vi "VIH HelpGen - Get Control Tag.vi"(7 "Separator (.)":string=".", 8 "error in":errorcluster, 9 "Skip Cluster if it's Array element (T)":bool=TRUE, 11 "Ctl Refnum":refnum<vi>) -> (0 "error out":errorcluster, 1 "Label":string, 2 "Control Tag":string, 3 "dup Ctl Refnum":refnum<vi>, 4 "Class Name":string, 5 "Parent Control Tag":string)   [LabVIEW 2014]
doc: "The VI builds a Control Tag of the specified control.\n\n::: VI Helpeks :::\nCopyright (c) 2000-2026 Konstantin Shifershteyn. All rights reserved."
panel:
  # "VI Helpeks\nCopyright (c) 2012-2026 Konstantin Shifershteyn"
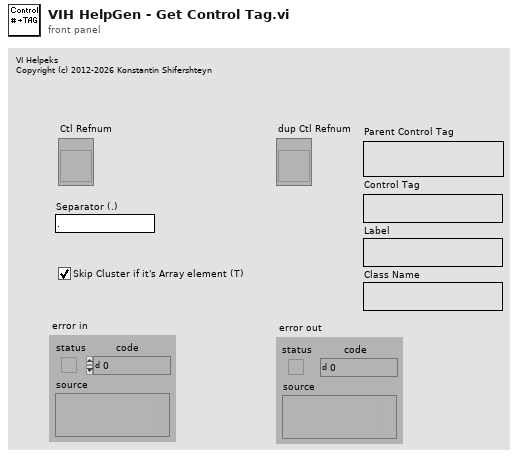
[diagram p1: front panel]
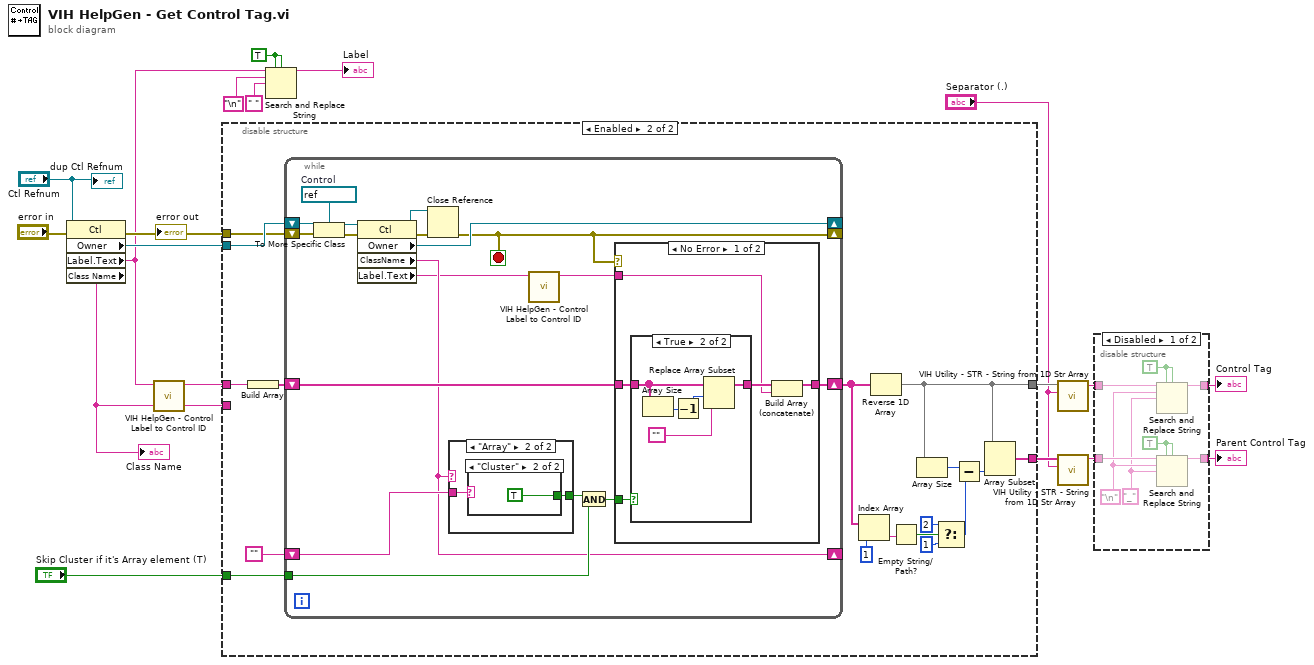
[diagram p0: block diagram]
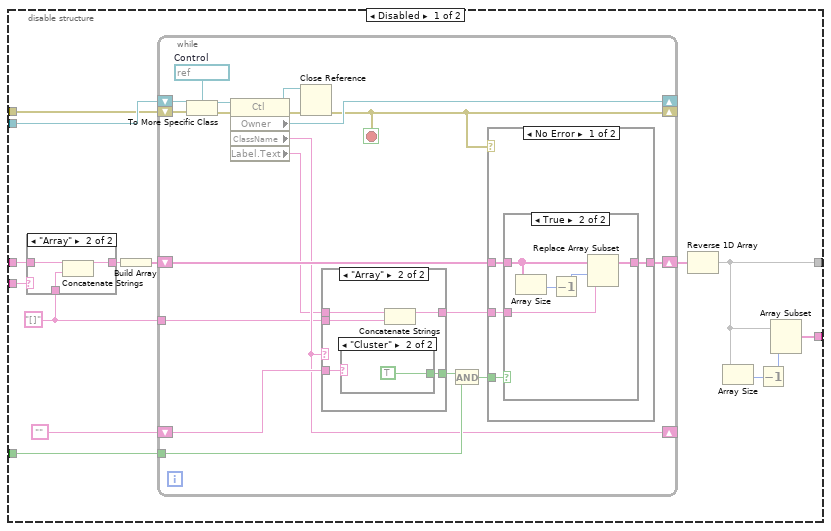
[diagram p3: hidden frame]
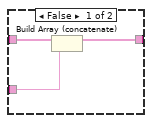
[diagram p7: hidden frame]
diagram:
  w5 = TRUE
  n1 = property class="Ctl"(reference="Ctl Refnum", error in="error in") -> (error out=w17:errorcluster, "Owner"=w18:refnum<vi>, "Label.Text"=w2:string, "Class Name"=w11:string)  [unwired: 1 out]
  "error out" <- w17
  "Class Name" <- w11
  n2 = call "VIH HelpGen - Control Label to Control ID.vi"("Control Name"=w2) -> ("Control ID"=w6:string)  [unwired: 10 in]
  n3 = disable-structure shown="Enabled" {
    disable-tunnel: w18 -> [w33 w93]
    disable-tunnel: w17 -> [w32 w92]
    disable-tunnel: "Skip Cluster if it's Array element (T)" -> [w30 w90]
    disable-tunnel: [w25 w77] -> w14
    disable-tunnel: [w24 w88] -> w13
    disable-tunnel: w6 -> [w23 w87]
    disable-tunnel: w11 -> [w20 _]
    frame Disabled {
      w21 = "[]" ("string")
      n4 = case shown="\"Array\"" w20 {
        tunnel: w23 -> [w34 w37]
        tunnel: [w34 w36] -> w22
        tunnel: w21 -> [_ w35]
        frame Default {
        }
        frame "Array" {
          n5 = Concatenate Strings(w37, w35) -> (w36:string)
        }
      }
      n6 = Build Array(w22) -> (w28:string[])
      n7 = while {
        shift-right: [w42] -> _
        shift-left: w32 -> [w49]
        shift-right: [w53] -> w29
        shift-left: w28 -> [w54]
        shift-right: [w52] -> _
        shift-left: w33 -> [w50]
        shift-right: [w43] -> _
        shift-left: "" -> [w45]
        tunnel: w30 -> [w44]
        tunnel: w21 -> [w38]
        stop <- w42 stop-if-true
        w51 = refnum<vi> refnum  # Control
        n8 = To More Specific Class(target class=w51, reference=w50, error in=w49) -> (specific class reference=w47:refnum<vi>, error out=w48:errorcluster)
        n9 = property class="Ctl"(reference=w47, error in=w48) -> (reference out=w56:refnum<vi>, error out=w55:errorcluster, "Owner"=w52:refnum<vi>, "ClassName"=w43:string, "Label.Text"=w41:string)
        n10 = Close Reference(reference=w56, error in (no error)=w55) -> (error out=w42:errorcluster)
        n11 = case shown="\"Array\"" w43 {
          tunnel: w45 -> [_ w62]
          tunnel: [_ w61] -> w46
          tunnel: w41 -> [w57 w60]
          tunnel: [w57 w59] -> w40
          tunnel: w38 -> [_ w58]
          frame Default {
          }
          frame "Array" {
            n12 = case shown="\"Cluster\"" w62 {
              tunnel: [_ TRUE] -> w61
              frame Default {
              }
              frame "Cluster" {
              }
            }
            n13 = Concatenate Strings(w60, w58) -> (w59:string)
          }
        }
        n14 = And(x=w46, y=w44) -> (x .and. y?=w39:bool)
        n15 = case shown="No Error" w42 {
          tunnel: w54 -> [w65 w76]
          tunnel: w40 -> [w67 _]
          tunnel: [w66 w76] -> w53
          tunnel: w39 -> [w64 _]
          frame No Error {
            n16 = case shown="True" w64 {
              tunnel: w67 -> [w69 w72]
              tunnel: [w68 w71] -> w66
              tunnel: w65 -> [w70 w75]
              frame False {
                n17 = Build Array (concatenate)(w70, w69) -> (w68:string[])
              }
              frame True {
                n18 = Array Size(array=w75) -> (size(s)=w74:i32)
                n19 = Decrement(x=w74) -> (x-1=w73:i32)
                n20 = Replace Array Subset(array=w75, new element=w72, index=w73) -> (w71:string[])
              }
            }
          }
          frame Error {
          }
        }
      }
      n21 = Reverse 1D Array(array=w29) -> (reversed array=w25:string[])
      n22 = Array Size(array=w25) -> (size(s)=w26:i32)
      n23 = Decrement(x=w26) -> (x-1=w27:i32)
      n24 = Array Subset(array=w25, length=w27) -> (w24:string[])  [unwired: 1 in]
    }
    frame Enabled {
      n25 = Build Array(w87) -> (w89:string[])
      n26 = while {
        shift-right: [w97] -> _
        shift-left: w92 -> [w104]
        shift-right: [w108] -> w82
        shift-left: w89 -> [w109]
        shift-right: [w107] -> _
        shift-left: w93 -> [w105]
        shift-right: [w98] -> _
        shift-left: "" -> [w100]
        tunnel: w90 -> [w99]
        stop <- w97 stop-if-true
        w106 = refnum<vi> refnum  # Control
        n27 = To More Specific Class(target class=w106, reference=w105, error in=w104) -> (specific class reference=w102:refnum<vi>, error out=w103:errorcluster)
        n28 = property class="Ctl"(reference=w102, error in=w103) -> (reference out=w111:refnum<vi>, error out=w110:errorcluster, "Owner"=w107:refnum<vi>, "ClassName"=w98:string, "Label.Text"=w95:string)
        n29 = Close Reference(reference=w111, error in (no error)=w110) -> (error out=w97:errorcluster)
        n30 = case shown="\"Array\"" w98 {
          tunnel: w100 -> [_ w113]
          tunnel: [_ w112] -> w101
          frame Default {
          }
          frame "Array" {
            n31 = case shown="\"Cluster\"" w113 {
              tunnel: [_ TRUE] -> w112
              frame Default {
              }
              frame "Cluster" {
              }
            }
          }
        }
        n32 = call "VIH HelpGen - Control Label to Control ID.vi"("Control Name"=w95) -> ("Control ID"=w94:string)  [unwired: 10 in]
        n33 = And(x=w101, y=w99) -> (x .and. y?=w96:bool)
        n34 = case shown="No Error" w97 {
          tunnel: w109 -> [w119 w126]
          tunnel: [w116 w126] -> w108
          tunnel: w96 -> [w118 _]
          tunnel: w94 -> [w115 _]
          frame No Error {
            n35 = case shown="True" w118 {
              tunnel: [w120 w122] -> w117
              tunnel: w119 -> [w120 w125]
              frame False {
              }
              frame True {
                n36 = Array Size(array=w125) -> (size(s)=w124:i32)
                n37 = Decrement(x=w124) -> (x-1=w123:i32)
                n38 = Replace Array Subset(array=w125, new element="", index=w123) -> (w122:string[])
              }
            }
            n39 = Build Array (concatenate)(w117, w115) -> (w116:string[])
          }
          frame Error {
          }
        }
      }
      n40 = Index Array(array=w82, index=1) -> (element=w80:string)
      n41 = Reverse 1D Array(array=w82) -> (reversed array=w77:string[])
      n42 = Empty String/Path?(string/path=w80) -> (empty?=w78:bool)
      n43 = Array Size(array=w77) -> (size(s)=w85:i32)
      n44 = Select(t=2, s=w78, f=1) -> (s? t:f=w83:i32)
      n45 = Subtract(x=w85, y=w83) -> (x-y=w86:i32)
      n46 = Array Subset(array=w77, length=w86) -> (w88:string[])  [unwired: 1 in]
    }
  }
  n47 = Search and Replace String(replace all?=w5, case sensitive?=w5, input string=w2, search string="\n", replace string=" " ("replace string (\"\")")) -> (result string=→"Label":string)  [unwired: 3 in, 3 out]
  n48 = call "VIH Utility - STR - String from 1D Str Array.vi"("delimiter ('\\n')"="Separator (.)", "Array in"=w14) -> ("String out"=w10:string)  [unwired: 5 in]
  n49 = call "VIH Utility - STR - String from 1D Str Array.vi"("delimiter ('\\n')"="Separator (.)", "Array in"=w13) -> ("String out"=w8:string)  [unwired: 5 in]
  n50 = disable-structure shown="Disabled" {
    disable-tunnel: w10 -> [w132 w136]
    disable-tunnel: [w131 w136] -> w9
    disable-tunnel: w8 -> [w130 w135]
    disable-tunnel: [w129 w135] -> w7
    frame Disabled {
      w127 = "_" ("replace string (\"\")")
      w133 = TRUE
      w128 = "\n"
      w134 = TRUE
      n51 = Search and Replace String(replace all?=w134, case sensitive?=w134, input string=w132, search string=w128, replace string=w127) -> (result string=w131:string)  [unwired: 3 in, 3 out]
      n52 = Search and Replace String(replace all?=w133, case sensitive?=w133, input string=w130, search string=w128, replace string=w127) -> (result string=w129:string)  [unwired: 3 in, 3 out]
    }
    frame Enabled {
    }
  }
  "Control Tag" <- w9
  "Parent Control Tag" <- w7
  "dup Ctl Refnum" <- "Ctl Refnum"
